vi "Temperature Controller Demo.vi"() -> ()   [LabVIEW 2021]
uses:
  Support/Demo Mode.ctl
  <vilib>/TSA/Omni-Bus/Omni-Bus/Omni_Bus.lvclass
  <vilib>/TSA/Omni-Bus/Omni-Bus/Support/Read/Read Boolean.vi
  <vilib>/TSA/Omni-Bus/Omni-Bus/Support/Read/Read DBL.vi
  <vilib>/TSA/Omni-Bus/Omni-Bus/Support/Write/Write Boolean.vi
  <vilib>/TSA/Omni-Bus/Omni-Bus/Support/Get/Get DBL.vi
  <vilib>/TSA/Omni-Bus/Omni-Bus/Support/Get/Get Boolean.vi
  <vilib>/TSA/Abstract Data Classes/Abs_Types/Boolean/Static Read.vi
  <vilib>/TSA/Abstract Data Classes/Abs_Types/Double Float/Static Read.vi
  <vilib>/TSA/Abstract Data Classes/Abs_Types/Boolean/Static Write.vi
  <vilib>/TSA/Abstract Data Classes/Abs_Types/Double Float/Simple Read.vi
  <vilib>/TSA/Abstract Data Classes/Abs_Types/Boolean/Simple Read.vi
  <vilib>/TSA/Abstract Data Classes/Abs_Types/Boolean/Abs_Boolean.lvclass
  C:/Program Files (x86)/National Instruments/LabVIEW 2021/vi.lib/TSA/Abstract Data Classes/Abs_Types/Type/Abs_Type.lvclass
  C:/Program Files (x86)/National Instruments/LabVIEW 2021/vi.lib/TSA/Abstract Data Classes/Abs_Types/Value/Abs_Value.lvclass
  <vilib>/TSA/Abstract Data Classes/Abs_Types/Double Float/Abs_Double Float.lvclass
  <vilib>/TSA/Omni-Bus/Omni-Bus/Support/FindVar.vi
  Support/Temperature Limits.vi
  <vilib>/TSA/Abstract Data Classes/Functions/Logic/Support/NOT/Bool/Method.vi
  <vilib>/TSA/Abstract Data Classes/Functions/Compare/Support/Less/DBL/Method_Const.vi
  <vilib>/TSA/Abstract Data Classes/Functions/Logic/Support/AND/Bool/Method.vi
  <vilib>/TSA/Abstract Data Classes/Functions/Logic/Support/OR/Bool/Method.vi
  <vilib>/TSA/Abstract Data Classes/Functions/Logic/Support/AND/Bool/AND_Bool.lvclass
  <vilib>/TSA/Abstract Data Classes/Functions/Logic/Support/NOT/Bool/NOT_Bool.lvclass
  <vilib>/TSA/Abstract Data Classes/Functions/Logic/Support/OR/Bool/OR_Bool.lvclass
  <vilib>/TSA/Abstract Data Classes/Functions/Compare/Support/Less/DBL/Less_DBL.lvclass
panel:
  in  "Algorthym":T1(ring)
  in  "Modes":T2
  out "Tags":i32(listbox)
  in  "Stop Button":bool
  out "Heater State":bool
  out "Temperature Chart":T3(graph)
  out "Temperature":dbl(knob) scale=10.0..90.0
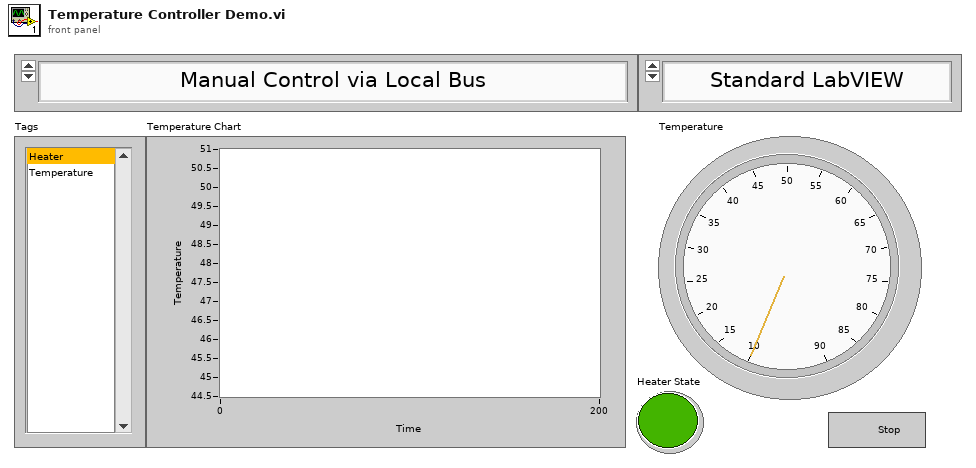
[diagram p1: front panel]
types:
  T1 = enum16{"Standard LabVIEW", "Object Read and Write", "Object Functional 1", "Object Functional 2"}
  T2 = typedef "Demo Mode.ctl" = enum16{"Manual Control via Local Bus", "Software In the Loop via Local Bus", "NI USB6001 DAQ via DAQmx - Without Aliasing", "NI USB6001 DAQ via DAQmx - With Aliasing", "NI cRIO FPGA via TCP", "Community Training Initiative Raspberry Pi Pico", "NI USB6001 DAQ via DAQmx with Fault Insertion", "Mixed Devices"}
  T3 = cluster{"Temperature":dbl, "Upper Temp":dbl, "Lower Temp":dbl}
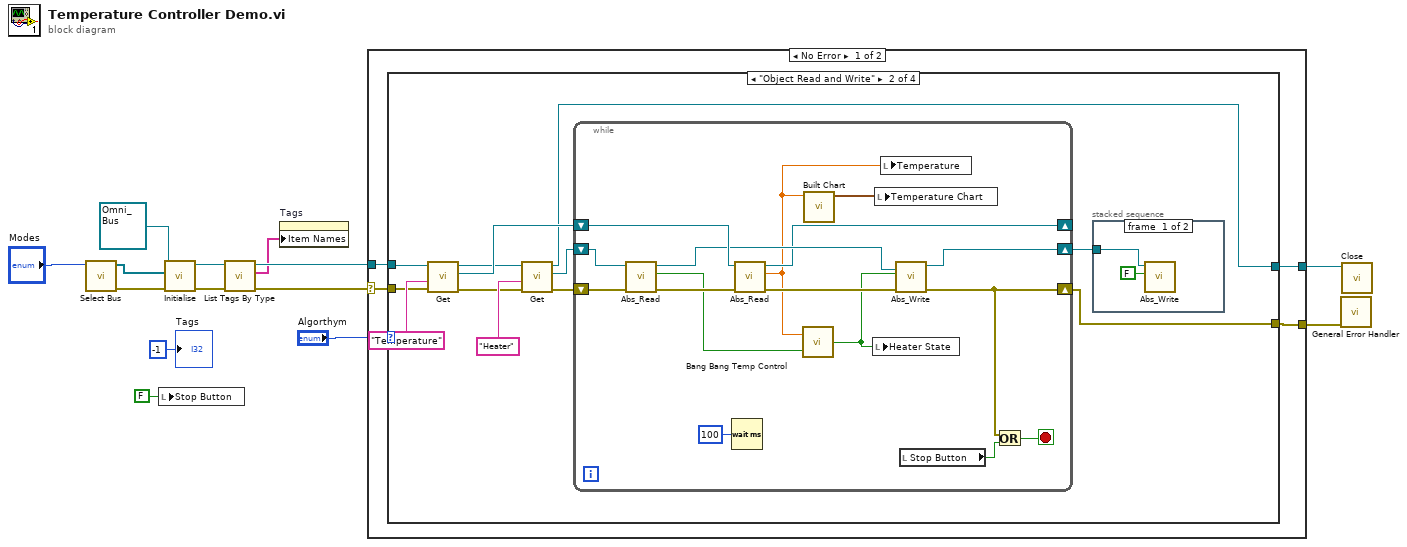
[diagram p0: block diagram]
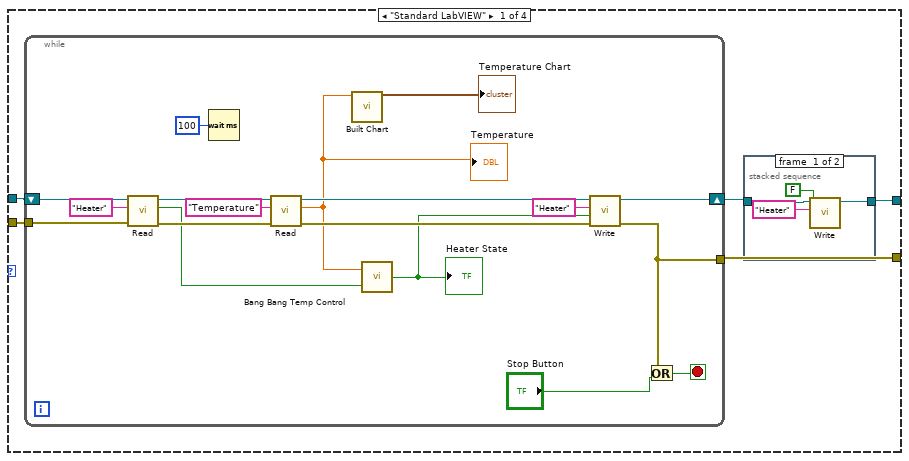
[diagram p2: hidden frame]
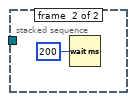
[diagram p3: hidden frame]
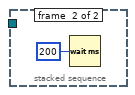
[diagram p4: hidden frame]
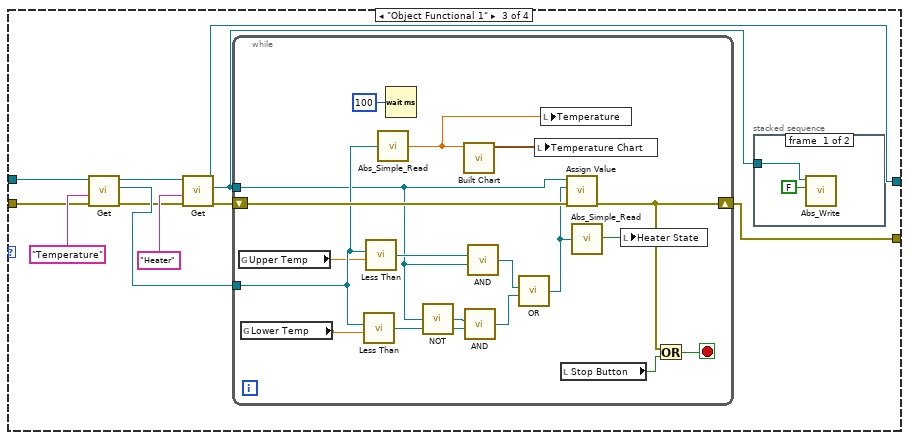
[diagram p5: hidden frame]
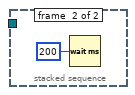
[diagram p6: hidden frame]
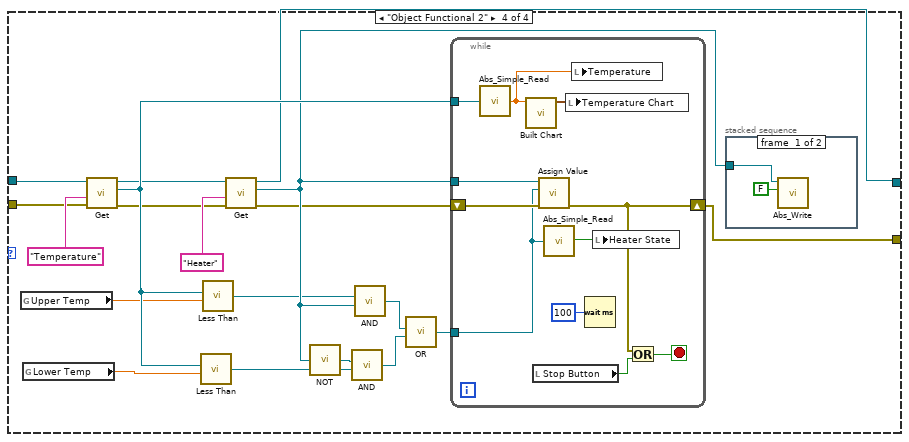
[diagram p7: hidden frame]
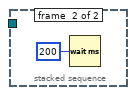
[diagram p8: hidden frame]
diagram:
  n1 = call "Select Bus.vi"("Modes"="Modes") -> ("error out"=w10:errorcluster, "Array"=w8:refnum<class "Bus_Access.lvclass">[])  [unwired: 9 in]
  n2 = local write "Stop Button"(FALSE ("Stop Button")) -> ()
  n3 = call-dynamic "Initialise.vi"("error in (no error)"=w10, "Bus Access"=w8, "Var Bus in"=refnum<class "Omni_Bus.lvclass"> refnum) -> ("error out"=w12:errorcluster, "Var Bus out"=w13:refnum<class "Omni_Bus.lvclass">)  [unwired: 7 in]
  n4 = call <vilib>:"List Tags By Type.vi"("error in (no error)"=w12, "Var Bus in"=w13) -> ("error out"=w7:errorcluster, "Tags"=w5:string[], "Var Bus out"=w11:refnum<class "Omni_Bus.lvclass">)  [unwired: 6 in, 1 out]
  n5 = property on="Tags" class="LstBox (strict)"("Item Names"=w5) -> ()  [unwired: 2 in, 2 out]
  n6 = case shown="No Error" w7 {
    selector: w7 -> [w16 w144]
    tunnel: [w18 w145] -> w14
    tunnel: w11 -> [w17 w145]
    tunnel: [w19 w144] -> w6
    tunnel: "Algorthym" -> [w15 _]
    frame No Error {
      n7 = case shown="\"Object Read and Write\"" w15 {
        tunnel: [w20 w48 w81 w111] -> w19
        tunnel: [w23 w49 w82 w112] -> w18
        tunnel: w17 -> [w22 w50 w80 w114]
        tunnel: w16 -> [w21 w51 w79 w113]
        frame "Standard LabVIEW" {
          n8 = while {
            shift-right: [w44] -> w24
            shift-left: w22 -> [w47]
            tunnel: [w36] -> w20
            tunnel: w21 -> [w30]
            stop <- w39 stop-if-true
            n9 = call-poly <vilib>:"Read.vi"("error in (no error)"=w30, "Tag"="Heater", "Var Bus in"=w47) -> ("error out"=w37:errorcluster, "Boolean"=w32:bool, "Var Bus out"=w46:refnum<class "Omni_Bus.lvclass">)  [unwired: 6 in]
            n10 = Wait (ms)(milliseconds to wait=u32 100) -> ()  [unwired: 1 out]
            n11 = call-poly <vilib>:"Read.vi"("error in (no error)"=w37, "Tag"="Temperature", "Var Bus in"=w46) -> ("error out"=w38:errorcluster, "Numeric"=w35:dbl, "Var Bus out"=w45:refnum<class "Omni_Bus.lvclass">)  [unwired: 6 in]
            "Temperature" <- w35
            n12 = call "Built Chart.vi"("Temperature"=w35) -> ("Chart"=→"Temperature Chart":T3)  [unwired: 6 in]
            n13 = call "Bang Bang Temp Control.vi"("Previous Heater State"=w32, "Temperature"=w35) -> ("New Heater State"=w31:bool)
            "Heater State" <- w31
            n14 = call-poly <vilib>:"Write.vi"("error in (no error)"=w38, "Boolean"=w31, "Tag"="Heater", "Omni_Bus in"=w45) -> ("error out"=w36:errorcluster, "Omni_Bus out"=w44:refnum<class "Omni_Bus.lvclass">)  [unwired: 6 in]
            n15 = Or(x=w36, y="Stop Button") -> (x .or. y?=w39:bool)
          }
          n16 = stacked-sequence {
            tunnel: w24 -> [w27 _]
            tunnel: [w26 _] -> w23
            frame #0 {
              n17 = call-poly <vilib>:"Write.vi"("Boolean"=FALSE, "Tag"="Heater", "Omni_Bus in"=w27) -> ("Omni_Bus out"=w26:refnum<class "Omni_Bus.lvclass">)  [unwired: 7 in, 1 out]
            }
            frame #1 {
              n18 = Wait (ms)(milliseconds to wait=u32 200) -> ()  [unwired: 1 out]
            }
          }
        }
        frame "Object Read and Write" {
          n19 = call-poly <vilib>:"Get.vi"("error in (no error)"=w51, "Tag"="Temperature", "Var Bus in"=w50) -> ("error out"=w53:errorcluster, "Value Out"=w54:refnum<class "Abs_Double Float.lvclass">, "Var Bus out"=w52:refnum<class "Omni_Bus.lvclass">)  [unwired: 5 in, 1 out]
          n20 = call-poly <vilib>:"Get.vi"("error in (no error)"=w53, "Tag"="Heater", "Var Bus in"=w52) -> ("error out"=w55:errorcluster, "Value Out"=w56:refnum<class "Abs_Boolean.lvclass">, "Var Bus out"=w49:refnum<class "Omni_Bus.lvclass">)  [unwired: 5 in, 1 out]
          n21 = while {
            shift-right: [w63] -> w48
            shift-left: w55 -> [w75]
            shift-right: [w70] -> _
            shift-left: w54 -> [w72]
            shift-right: [w73] -> w58
            shift-left: w56 -> [w74]
            stop <- w77 stop-if-true
            n22 = call-poly <vilib>:"Abs_Read.vi"("error in (no error)"=w75, "Abs_Boolean in"=w74) -> ("error out"=w69:errorcluster, "Boolean"=w67:bool, "Abs_Boolean out"=w71:refnum<class "Abs_Boolean.lvclass">)  [unwired: 7 in]
            n23 = Wait (ms)(milliseconds to wait=u32 100) -> ()  [unwired: 1 out]
            n24 = call-poly <vilib>:"Abs_Read.vi"("error in (no error)"=w69, "Abs_Double Float in"=w72) -> ("error out"=w68:errorcluster, "Value"=w65:dbl, "Abs_Double Float out"=w70:refnum<class "Abs_Double Float.lvclass">)  [unwired: 7 in]
            n25 = call "Bang Bang Temp Control.vi"("Previous Heater State"=w67, "Temperature"=w65) -> ("New Heater State"=w64:bool)
            n26 = call "Built Chart.vi"("Temperature"=w65) -> ("Chart"=w66:T3)  [unwired: 6 in]
            n27 = local write "Heater State"(w64) -> ()
            n28 = local write "Temperature Chart"(w66) -> ()
            n29 = local write "Temperature"(w65) -> ()
            n30 = call-poly <vilib>:"Abs_Write.vi"("error in (no error)"=w68, "Boolean"=w64, "Abs_Boolean in"=w71) -> ("error out"=w63:errorcluster, "Abs_Boolean out"=w73:refnum<class "Abs_Boolean.lvclass">)  [unwired: 7 in]
            n31 = local read "Stop Button"() -> (w76:bool)
            n32 = Or(x=w63, y=w76) -> (x .or. y?=w77:bool)
          }
          n33 = stacked-sequence {
            tunnel: w58 -> [w61 _]
            frame #0 {
              n34 = call-poly <vilib>:"Abs_Write.vi"("Boolean"=FALSE, "Abs_Boolean in"=w61) -> ()  [unwired: 8 in, 2 out]
            }
            frame #1 {
              n35 = Wait (ms)(milliseconds to wait=u32 200) -> ()  [unwired: 1 out]
            }
          }
        }
        frame "Object Functional 1" {
          n36 = call-poly <vilib>:"Get.vi"("error in (no error)"=w79, "Tag"="Temperature", "Var Bus in"=w80) -> ("error out"=w84:errorcluster, "Value Out"=w88:refnum<class "Abs_Double Float.lvclass">, "Var Bus out"=w83:refnum<class "Omni_Bus.lvclass">)  [unwired: 5 in, 1 out]
          n37 = call-poly <vilib>:"Get.vi"("error in (no error)"=w84, "Tag"="Heater", "Var Bus in"=w83) -> ("error out"=w85:errorcluster, "Value Out"=w89:refnum<class "Abs_Boolean.lvclass">, "Var Bus out"=w82:refnum<class "Omni_Bus.lvclass">)  [unwired: 5 in, 1 out]
          n38 = while {
            shift-right: [w101] -> w81
            shift-left: w85 -> [w100]
            tunnel: w88 -> [w97]
            tunnel: w89 -> [w95]
            stop <- w109 stop-if-true
            n39 = global read "Temperature Limits.vi" "Upper Temp"() -> (w94:dbl)
            n40 = global read "Temperature Limits.vi" "Lower Temp"() -> (w93:dbl)
            n41 = call-poly <vilib>:"Less Than.vi"("Value"=w93, "Value A"=w97) -> ("Result"=w102:refnum<class "Abs_Boolean.lvclass">)  [unwired: 4 in]
            n42 = call-poly <vilib>:"Less Than.vi"("Value"=w94, "Value A"=w97) -> ("Result"=w106:refnum<class "Abs_Boolean.lvclass">)  [unwired: 4 in]
            n43 = call-poly <vilib>:"Abs_Simple_Read.vi"("Class"=w97) -> ("Value"=w96:dbl)  [unwired: 4 in]
            n44 = Wait (ms)(milliseconds to wait=u32 100) -> ()  [unwired: 1 out]
            n45 = call-poly <vilib>:"NOT.vi"("Bool"=w95) -> ("Result"=w103:refnum<class "Abs_Boolean.lvclass">)  [unwired: 4 in]
            n46 = call "Built Chart.vi"("Temperature"=w96) -> ("Chart"=w107:T3)  [unwired: 6 in]
            n47 = call-poly <vilib>:"AND.vi"("B"=w102, "A"=w103) -> ("Result"=w105:refnum<class "Abs_Boolean.lvclass">)  [unwired: 4 in]
            n48 = call-poly <vilib>:"AND.vi"("B"=w95, "A"=w106) -> ("Result"=w104:refnum<class "Abs_Boolean.lvclass">)  [unwired: 4 in]
            n49 = call-poly <vilib>:"OR.vi"("B"=w105, "A"=w104) -> ("Result"=w99:refnum<class "Abs_Boolean.lvclass">)  [unwired: 4 in]
            n50 = local write "Temperature Chart"(w107) -> ()
            n51 = local write "Temperature"(w96) -> ()
            n52 = local read "Stop Button"() -> (w108:bool)
            n53 = call-dynamic "Assign Value.vi"("error in (no error)"=w100, "Assigned Value"=w99, "Abs_Boolean in"=w95) -> ("error out"=w101:errorcluster)  [unwired: 7 in, 1 out]
            n54 = call-poly <vilib>:"Abs_Simple_Read.vi"("Boolean in"=w99) -> ("Boolean"=w98:bool)  [unwired: 4 in]
            n55 = local write "Heater State"(w98) -> ()
            n56 = Or(x=w101, y=w108) -> (x .or. y?=w109:bool)
          }
          n57 = stacked-sequence {
            tunnel: w89 -> [w91 _]
            frame #0 {
              n58 = call-poly <vilib>:"Abs_Write.vi"("Boolean"=FALSE, "Abs_Boolean in"=w91) -> ()  [unwired: 8 in, 2 out]
            }
            frame #1 {
              n59 = Wait (ms)(milliseconds to wait=u32 200) -> ()  [unwired: 1 out]
            }
          }
        }
        frame "Object Functional 2" {
          n60 = global read "Temperature Limits.vi" "Upper Temp"() -> (w125:dbl)
          n61 = global read "Temperature Limits.vi" "Lower Temp"() -> (w126:dbl)
          n62 = call-poly <vilib>:"Get.vi"("error in (no error)"=w113, "Tag"="Temperature", "Var Bus in"=w114) -> ("error out"=w116:errorcluster, "Value Out"=w129:refnum<class "Abs_Double Float.lvclass">, "Var Bus out"=w115:refnum<class "Omni_Bus.lvclass">)  [unwired: 5 in, 1 out]
          n63 = call-poly <vilib>:"Less Than.vi"("Value"=w126, "Value A"=w129) -> ("Result"=w124:refnum<class "Abs_Boolean.lvclass">)  [unwired: 4 in]
          n64 = call-poly <vilib>:"Less Than.vi"("Value"=w125, "Value A"=w129) -> ("Result"=w120:refnum<class "Abs_Boolean.lvclass">)  [unwired: 4 in]
          n65 = call-poly <vilib>:"Get.vi"("error in (no error)"=w116, "Tag"="Heater", "Var Bus in"=w115) -> ("error out"=w117:errorcluster, "Value Out"=w128:refnum<class "Abs_Boolean.lvclass">, "Var Bus out"=w112:refnum<class "Omni_Bus.lvclass">)  [unwired: 5 in, 1 out]
          n66 = call-poly <vilib>:"NOT.vi"("Bool"=w128) -> ("Result"=w123:refnum<class "Abs_Boolean.lvclass">)  [unwired: 4 in]
          n67 = call-poly <vilib>:"AND.vi"("B"=w124, "A"=w123) -> ("Result"=w121:refnum<class "Abs_Boolean.lvclass">)  [unwired: 4 in]
          n68 = call-poly <vilib>:"AND.vi"("B"=w128, "A"=w120) -> ("Result"=w122:refnum<class "Abs_Boolean.lvclass">)  [unwired: 4 in]
          n69 = call-poly <vilib>:"OR.vi"("B"=w121, "A"=w122) -> ("Result"=w127:refnum<class "Abs_Boolean.lvclass">)  [unwired: 4 in]
          n70 = while {
            shift-right: [w139] -> w111
            shift-left: w117 -> [w138]
            tunnel: w128 -> [w135]
            tunnel: w127 -> [w134]
            tunnel: w129 -> [w133]
            stop <- w142 stop-if-true
            n71 = call-poly <vilib>:"Abs_Simple_Read.vi"("Class"=w133) -> ("Value"=w136:dbl)  [unwired: 4 in]
            n72 = call "Built Chart.vi"("Temperature"=w136) -> ("Chart"=w140:T3)  [unwired: 6 in]
            n73 = local read "Stop Button"() -> (w141:bool)
            n74 = call-dynamic "Assign Value.vi"("error in (no error)"=w138, "Assigned Value"=w134, "Abs_Boolean in"=w135) -> ("error out"=w139:errorcluster)  [unwired: 7 in, 1 out]
            n75 = call-poly <vilib>:"Abs_Simple_Read.vi"("Boolean in"=w134) -> ("Boolean"=w137:bool)  [unwired: 4 in]
            n76 = local write "Temperature Chart"(w140) -> ()
            n77 = local write "Temperature"(w136) -> ()
            n78 = Wait (ms)(milliseconds to wait=u32 100) -> ()  [unwired: 1 out]
            n79 = local write "Heater State"(w137) -> ()
            n80 = Or(x=w139, y=w141) -> (x .or. y?=w142:bool)
          }
          n81 = stacked-sequence {
            tunnel: w128 -> [w131 _]
            frame #0 {
              n82 = call-poly <vilib>:"Abs_Write.vi"("Boolean"=FALSE, "Abs_Boolean in"=w131) -> ()  [unwired: 8 in, 2 out]
            }
            frame #1 {
              n83 = Wait (ms)(milliseconds to wait=u32 200) -> ()  [unwired: 1 out]
            }
          }
        }
      }
    }
    frame Error {
    }
  }
  n84 = call <vilib>:"General Error Handler.vi"("error in (no error)"=w6) -> ()  [unwired: 10 in, 5 out]
  n85 = call-dynamic "Close.vi"("Data in"=w14) -> ()  [unwired: 9 in, 2 out]
  "Tags" <- -1 ("Tags")
